vi "List Rules as Strings.vi"(8 "error in (no error)":errorcluster, 11 "GlobalLogFilter In":refnum<class "LogFilter.lvclass">) -> (0 "error out":errorcluster, 2 "Rule Strings":string[](array[string]), 3 "GlobalLogFilter Out":refnum<class "LogFilter.lvclass">)   [LabVIEW 2017, in "CSM File Logger.lvlib"]
doc: "### List Rules as Strings.vi\n\n-- <b>Controls</b> --\n- <b>GlobalLogFilter in</b>:\n\n-- <b>Indicators</b> --\n- <b>Rule Strings</b>:\n- <b>GlobalLogFilter out</b>:"
uses:
  CSM File Logger.lvlib
  _Support/GlobalEvent/LogFilter/LogFilter.lvclass
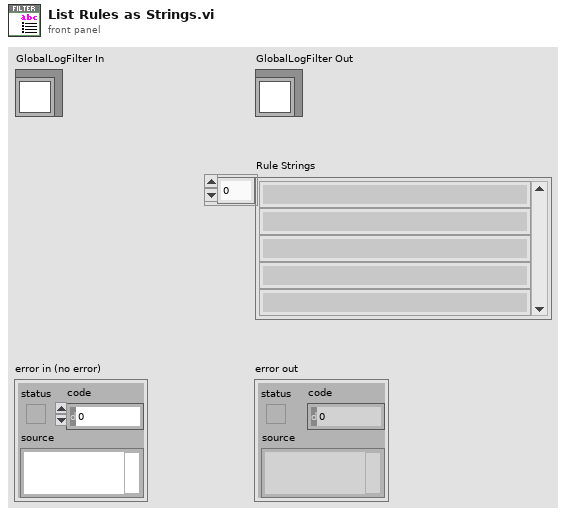
[diagram p1: front panel]
types:
  T1 = typedef "Communicable State Machine.lvlib/_CSM_GlobalLog_MSG_TYPE.ctl" = enum16{"User Log", "State Change", "Status", "Interrupt", "Register", "Unregister", "Error Log", "Module Created", "Module Destroyed"}
  T2 = typedef "Communicable State Machine.lvlib/_CSM_GlobalLog_STATE_TYPE.ctl" = enum16{"State - Internal State", "State - External Message", "State - Response", "State - Complete"}
  T3 = cluster{"Global":cluster{"CSM":string[], "LogType":T1[], "State":string[], "StateType":T2[]}, "CSM":cluster{"LogType":cluster{"CSM":string, "LogType":T1}[], "State":cluster{"CSM":string, "State":string}[], "StateType":cluster{"CSM":string, "LogType":T2}[]}, "PeriodicLog":cluster{"Enable":bool, "Threshold(#/s)":dbl, "CheckPeriod(s)":dbl}}
  T4 = cluster{"Enable":bool, "Threshold(#/s)":dbl, "CheckPeriod(s)":dbl}
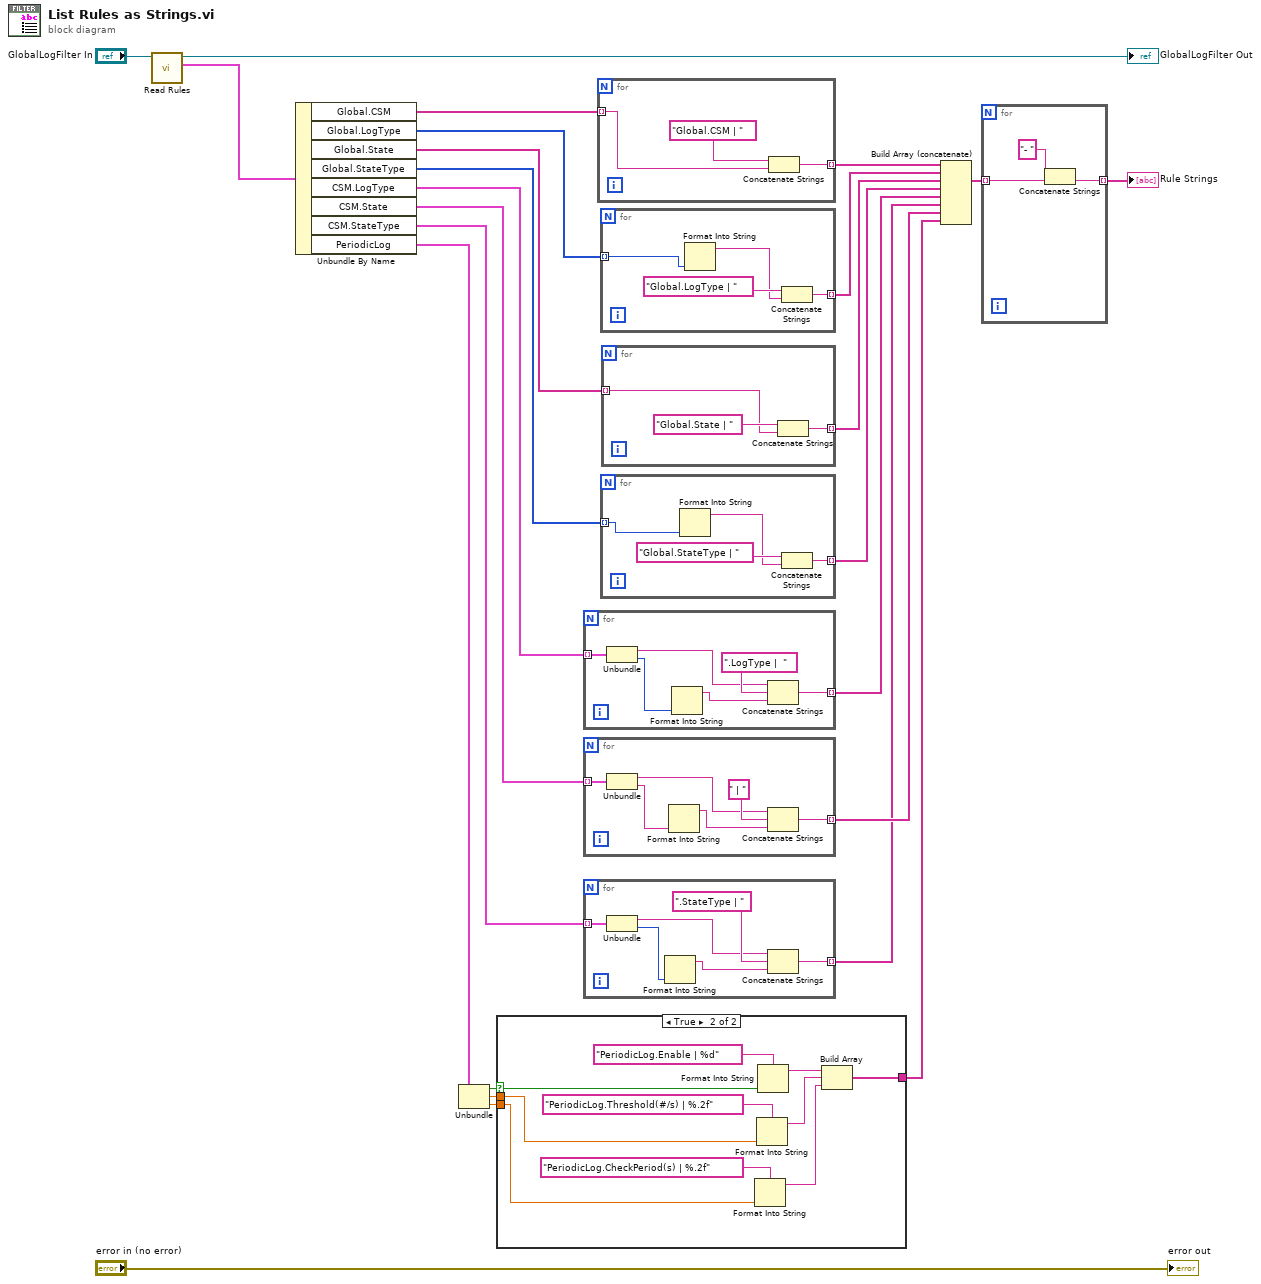
[diagram p0: block diagram]
diagram:
  n1 = call "Read Rules.vi"("LogFilter In"="GlobalLogFilter In") -> ("Rules"=w6:T3, "LogFilter Out"=→"GlobalLogFilter Out":refnum<class "LogFilter.lvclass">)  [unwired: 8 in, 1 out]
  n2 = Unbundle By Name(w6) -> ("Global.CSM"=w23:string[], "Global.LogType"=w21:T1[], "Global.State"=w19:string[], "Global.StateType"=w11:T2[], "CSM.LogType"=w17:cluster{"CSM":string, "LogType":T1}[], "CSM.State"=w15:cluster{"CSM":string, "State":string}[], "CSM.StateType"=w9:cluster{"CSM":string, "LogType":T2}[], "PeriodicLog"=w5:T4)
  n3 = Unbundle(w5) -> ("Enable"=w4:bool, "Threshold(#/s)"=w3:dbl, "CheckPeriod(s)"=w2:dbl)
  n4 = case shown="True" w4 {
    selector: w4 -> [_ w35]
    tunnel: w3 -> [_ w32]
    tunnel: w2 -> [_ w30]
    tunnel: [_ w26] -> w1
    frame False {
    }
    frame True {
      n5 = Format Into String(format string="PeriodicLog.CheckPeriod(s) | %.2f", w30) -> (resulting string=w27:string)  [unwired: 2 in, 1 out]
      n6 = Format Into String(format string="PeriodicLog.Threshold(#/s) | %.2f", w32) -> (resulting string=w28:string)  [unwired: 2 in, 1 out]
      n7 = Format Into String(format string="PeriodicLog.Enable | %d", w35) -> (resulting string=w29:string)  [unwired: 2 in, 1 out]
      n8 = Build Array(w29, w28, w27) -> (w26:string[])
    }
  }
  n9 = for {
    tunnel: w17 -> [w39] mode=indexing
    tunnel: [w40] -> w16 mode=indexing
    n10 = Unbundle(w39) -> ("CSM"=w38:string, "LogType"=w37:T1)
    n11 = Format Into String(w37) -> (resulting string=w36:string)  [unwired: 3 in, 1 out]
    n12 = Concatenate Strings(w38, ".LogType |  " ("string"), w36) -> (w40:string)
  }
  n13 = for {
    tunnel: w15 -> [w45] mode=indexing
    tunnel: [w46] -> w14 mode=indexing
    n14 = Unbundle(w45) -> ("CSM"=w44:string, "State"=w43:string)
    n15 = Format Into String(w43) -> (resulting string=w42:string)  [unwired: 3 in, 1 out]
    n16 = Concatenate Strings(w44, " | " ("string"), w42) -> (w46:string)
  }
  n17 = for {
    tunnel: w9 -> [w51] mode=indexing
    tunnel: [w52] -> w8 mode=indexing
    n18 = Unbundle(w51) -> ("CSM"=w50:string, "LogType"=w49:T2)
    n19 = Format Into String(w49) -> (resulting string=w48:string)  [unwired: 3 in, 1 out]
    n20 = Concatenate Strings(w50, ".StateType | " ("string"), w48) -> (w52:string)
  }
  n21 = for {
    tunnel: w23 -> [w55] mode=indexing
    tunnel: [w54] -> w22 mode=indexing
    n22 = Concatenate Strings("Global.CSM | " ("string"), w55) -> (w54:string)
  }
  n23 = for {
    tunnel: w21 -> [w58] mode=indexing
    tunnel: [w59] -> w20 mode=indexing
    n24 = Format Into String(w58) -> (resulting string=w57:string)  [unwired: 3 in, 1 out]
    n25 = Concatenate Strings("Global.LogType | " ("string"), w57) -> (w59:string)
  }
  n26 = for {
    tunnel: w11 -> [w62] mode=indexing
    tunnel: [w63] -> w10 mode=indexing
    n27 = Format Into String(w62) -> (resulting string=w61:string)  [unwired: 3 in, 1 out]
    n28 = Concatenate Strings("Global.StateType | " ("string"), w61) -> (w63:string)
  }
  n29 = for {
    tunnel: w19 -> [w65] mode=indexing
    tunnel: [w66] -> w18 mode=indexing
    n30 = Concatenate Strings("Global.State | " ("string"), w65) -> (w66:string)
  }
  n31 = Build Array (concatenate)(w22, w20, w18, w10, w16, w8, w14, w1) -> (w12:string[])
  n32 = for {
    tunnel: [w68] -> w13 mode=indexing
    tunnel: w12 -> [w69] mode=indexing
    n33 = Concatenate Strings("- " ("string"), w69) -> (w68:string)
  }
  "Rule Strings" <- w13
  "error out" <- "error in (no error)"
